vi "Init.vi"(8 "error in (no error)":errorcluster, 10 "ID":string, 11 "Mixer in":refnum<class "Mixer.lvclass">) -> (0 "error out":errorcluster, 3 "Mixer out":refnum<class "Mixer.lvclass">)   [LabVIEW 2019, in "Mixer.lvclass"]
uses:
  Mixer.lvclass
  Packed Libraries/Audio Processing.lvlibp/Value Cluster.ctl
  Packed Libraries/Audio Processing.lvlibp/Value Properties.ctl
  Mixer.lvclass/Mixer.ctl
  Packed Libraries/Messaging.lvlibp
  Packed Libraries/Audio Processing.lvlibp
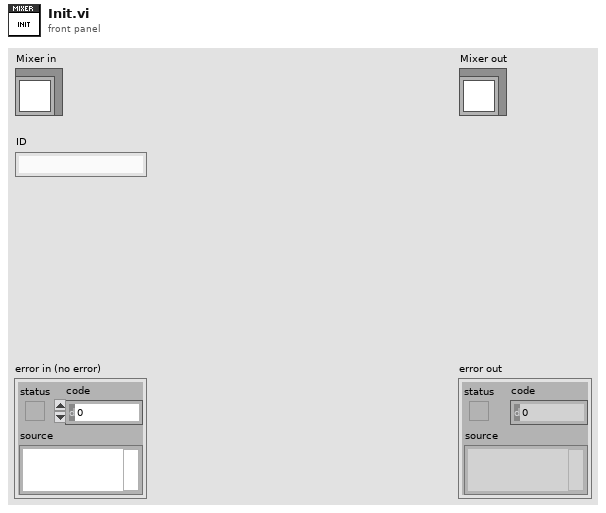
[diagram p1: front panel]
types:
  T1 = typedef "Audio Processing.lvlibp/Value Cluster.ctl" = cluster{"Value":dbl, "Properties":T2}
  T2 = typedef "Audio Processing.lvlibp/Value Properties.ctl" = cluster{"Lower":dbl, "Upper":dbl, "Default":dbl, "Increment":dbl}
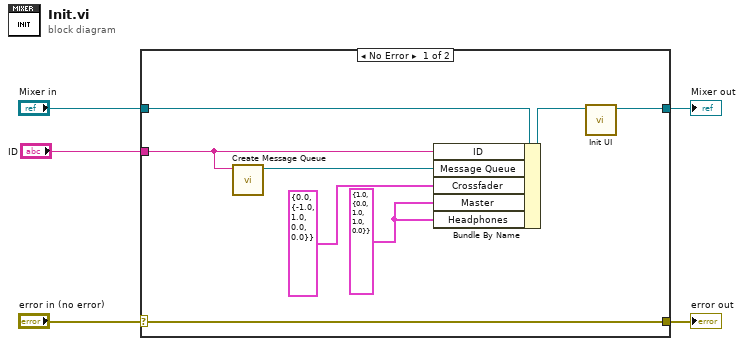
[diagram p0: block diagram]
diagram:
  n1 = case shown="No Error" "error in (no error)" {
    selector: "error in (no error)" -> [w13 w15]
    tunnel: [w13 w15] -> w4
    tunnel: [w6 w14] -> w2
    tunnel: "Mixer in" -> [w12 w14]
    tunnel: "ID" -> [w11 _]
    frame No Error {
      w9 = T1 {"Value"=1.0, "Properties"={"Lower"=0.0, "Upper"=1.0, "Default"=1.0, "Increment"=0.0}} ("Crossfader")
      n2 = call "Create Message Queue.vi"("Queue Name"=w11) -> ("queue out"=w10:refnum<queue>)  [unwired: 9 in, 1 out]
      n3 = Bundle By Name(cluster=w12, "ID"=w11, "Message Queue"=w10, "Crossfader"=T1 {"Value"=0.0, "Properties"={"Lower"=-1.0, "Upper"=1.0, "Default"=0.0, "Increment"=0.0}}, "Master"=w9, "Headphones"=w9) -> (w7:refnum<class "Mixer.lvclass">)
      n4 = call "Init UI.vi"("Mixer in"=w7) -> ("Mixer out"=w6:refnum<class "Mixer.lvclass">)  [unwired: 9 in, 1 out]
    }
    frame Error {
    }
  }
  "error out" <- w4
  "Mixer out" <- w2
